vi "Parse Params.vi"(8 "error in (no error)":errorcluster, 9 "<JSON> Params":string) -> (0 "error out":errorcluster, 1 "Params":string[](array[string]), 2 "Names":string[](array[string]))   [LabVIEW 2019, in "JSON-RPC.lvlib"]
uses:
  JSON-RPC.lvlib
  <vilib>/JDP Science/JSONtext/Get Array Elements.vi
  <vilib>/JDP Science/JSONtext/Get all Object Items.vi
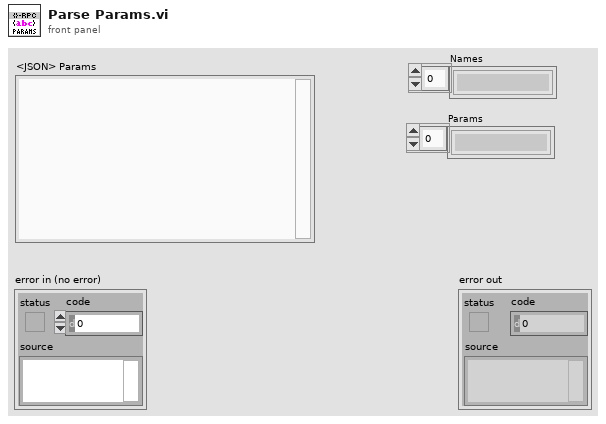
[diagram p1: front panel]
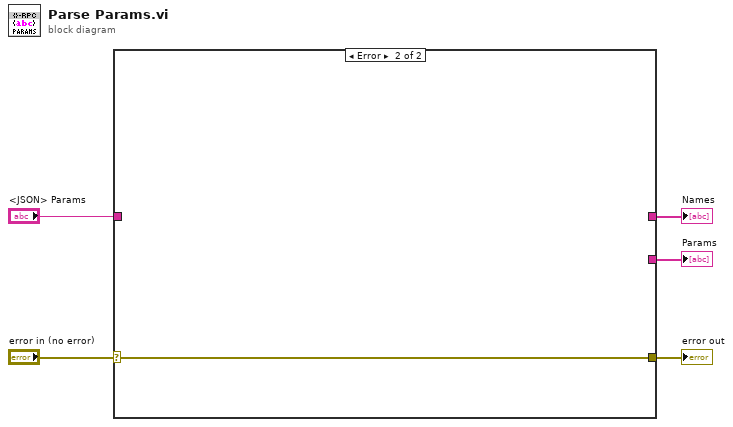
[diagram p0: block diagram]
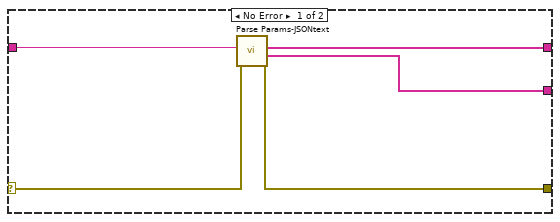
[diagram p2: hidden frame]
diagram:
  n1 = case shown="Error" "error in (no error)" {
    selector: "error in (no error)" -> [w9 w11]
    tunnel: [w8 w11] -> w4
    tunnel: "<JSON> Params" -> [w10 _]
    tunnel: [w7 _] -> w1
    tunnel: [w6 _] -> w2
    frame No Error {
      n2 = call "Parse Params-JSONtext.vi"("error in (no error)"=w9, "<JSON> params"=w10) -> ("error out"=w8:errorcluster, "Params"=w7:string[], "Names"=w6:string[])  [unwired: 7 in]
    }
    frame Error {
    }
  }
  "error out" <- w4
  "Names" <- w2
  "Params" <- w1
